vi "ZM-ROOT-createEvents.vi"(8 "error in (no error)":errorcluster, 11 "ZM-ROOT-root in":refnum<class "ZM-ROOT-root.lvclass">) -> (0 "error out":errorcluster, 3 "ZM-ROOT-root out":refnum<class "ZM-ROOT-root.lvclass">)   [LabVIEW 2020, in "ZM-ROOT-root.lvlib" / "ZM-ROOT-root.lvclass"]
doc: "Creates the root's stop and error user events and stores them in the events field (ZM-ROOT-EVENTS). Called by ZM-ROOT-createResources; the error goes out so a failed create fails the launch."
uses:
  ZM-ROOT-root.lvclass
  ZM-ROOT-root.lvclass/ZM-ROOT-root.ctl
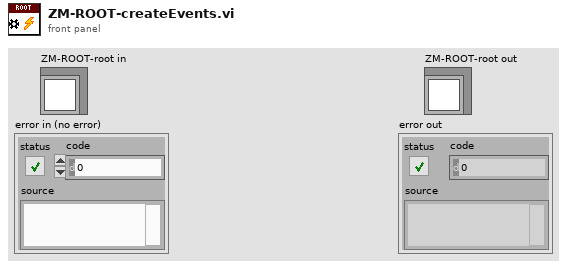
[diagram p1: front panel]
types:
  T1 = typedef "ZM-ROOT-root.lvlib/ZM-ROOT-root.lvclass/ZM-ROOT-EVENTS.ctl" = cluster{"stop":refnum<user-event>, "error":refnum<user-event>}
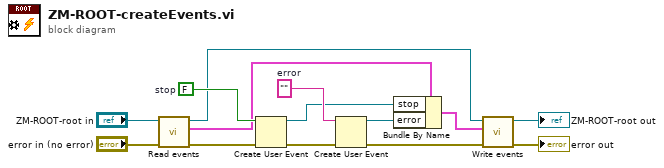
[diagram p0: block diagram]
diagram:
  w10 = ""  # error
  w12 = FALSE  # stop
  n1 = call "Read events.vi"("error in (no error)"="error in (no error)", "ZM-ROOT-root in"="ZM-ROOT-root in") -> ("error out"=w11:errorcluster, "ZM-ROOT-EVENTS"=w6:T1, "ZM-ROOT-root out"=w4:refnum<class "ZM-ROOT-root.lvclass">)  [unwired: 7 in]
  n2 = Create User Event(user event datatype=w12, error in=w11) -> (user event=w8:refnum<user-event>, error out=w9:errorcluster)
  n3 = Create User Event(user event datatype=w10, error in=w9) -> (user event=w7:refnum<user-event>, error out=w5:errorcluster)
  n4 = Bundle By Name(cluster=w6, "stop"=w8, "error"=w7) -> (w3:T1)
  n5 = call "Write events.vi"("error in (no error)"=w5, "ZM-ROOT-EVENTS"=w3, "ZM-ROOT-root in"=w4) -> ("error out"=→"error out":errorcluster, "ZM-ROOT-root out"=→"ZM-ROOT-root out":refnum<class "ZM-ROOT-root.lvclass">)  [unwired: 7 in]
